vi "editDialog.vi"(0 "reference":refnum<class "ClassNode.lvclass">, 1 "insidePackageNode":bool, 5 "error in (no error)":errorcluster) -> (14 "reference out":refnum<class "ClassNode.lvclass">, 15 "changeConnection":T2, 16 "cancel":bool, 19 "error out":errorcluster)   [LabVIEW 2020, in "ClassNode.lvclass"]
doc: "Edit Dialog"
uses:
  <resource>/Framework/Providers/Open_GDS/UML/ClassNode_class/ClassNode.lvclass
  C:/Program Files (x86)/National Instruments/LabVIEW 2020/resource/Framework/Providers/Open_GDS/UML/AbstractNode_class/AbstractNode.lvclass
  <resource>/Framework/Providers/Open_GDS/UML/AbstractNode_class/private/NodeConnectionStatsType.ctl
  <resource>/Framework/Providers/Open_GDS/UML/UMLEditor/UMLEditor_StoredPathes.ctl
  <resource>/Framework/Providers/Open_GDS/ClassProviders/Common/CommonVIs/CommonVIs_StereoType.ctl
  <resource>/Framework/Providers/Open_GDS/UML/ContextHelp/ContextHelp_HelpTexts.ctl
  <resource>/Framework/Providers/Open_GDS/UML/MultiLineString_class/MultiLineString.lvclass
  <resource>/Framework/Providers/Open_GDS/UML/AbstractNode_class/AbstractNode.lvclass
  <resource>/Framework/Providers/Open_GDS/UML/Graph_class/Graph.lvclass
panel:
  in  "Class owner":u16(ring) items=["<No owner>"]
  out "RelText":string="Relative path used"
  out "UserText":string="When creating an enum-type just state the different enumeration members in a list like this:\nE.g.\nElement 1\nElement 2\n\nE.g.\nVolt(V)\nCurrent(A)\nResistance(ohm)\n"
  in  "ShowAttrib":bool caption="Show Attributes"
  in  "ShowMethods":bool caption="Show Methods"
  in  "Help":bool
  in  "AddMethod":bool
  in  "AddAttribute":bool
  in  "Stereo Type":T1(ring)=enum."ENUM"
  in  "Class Name":string
  in  "ClassPath":path caption="LvClassPath(Optional)"
  in  "Attribute":string
  in  "Methods":string
  in  "connection":bool caption="Connect to Package"
  in  "Cancel Button":bool
  in  "OK Button":bool
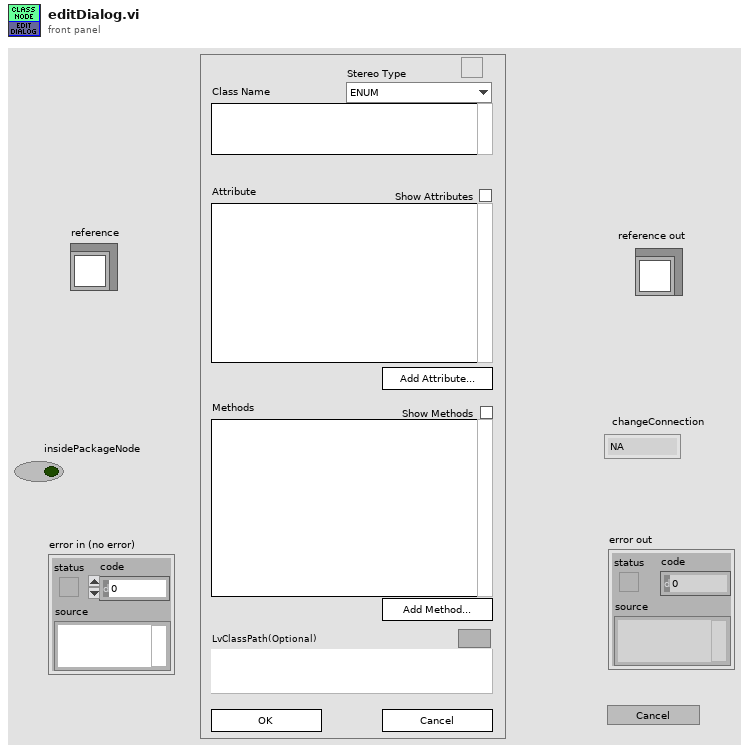
[diagram p1: front panel]
types:
  T1 = enum16{"None", "TYPE", "ENUM", "ABSTRACT", "ACTOR", "GUI", "SINGLETON", "SIGNAL", "BOUNDARY", "ENTITY", "CONTROL", "LEGACY", "APPLICATION", "VI", "LVLIB"}
  T2 = typedef "AbstractNode.lvclass/NodeConnectionStatsType.ctl" = enum16{"NA", "Connect", "DisConnect"}
  T3 = typedef "CommonVIs_StereoType.ctl" = enum16{"None", "TYPE", "ENUM", "ABSTRACT", "ACTOR", "GUI", "SINGLETON", "SIGNAL", "BOUNDARY", "ENTITY", "CONTROL", "LEGACY", "APPLICATION", "VI", "LVLIB", "INTERFACE"}
  T4 = typedef "UMLEditor_StoredPathes.ctl" = enum16{"LastSearchPath", "QueuedArrayStateVI", "ClassBasePath", "ViTemplatePath", "ApplicationTemplatePath", "IniFilePath", "WizDir", "RevPlugInPath"}
  T5 = enum32{"existing file", "new file", "new or existing file", "existing dir", "new dir", "new or existing dir", "existing file (use LLBs)", "new file (use LLBs)", "new or existing file (use LLBs)", "new or existing file or directory (use LLBs)"}
  T6 = enum16{"None", "TYPE", "ENUM", "GUI", "SINGLETON", "SIGNAL", "BOUNDARY", "ENTITY", "CONTROL", "LEGACY", "APPLICATION", "VI", "LVLIB"}
  T7 = typedef "ContextHelp_HelpTexts.ctl" = enum16{"None(Hide)", "Default", "Help", "Welcome", "GettingStarted", "ClassDiagram_Help", "SequenceDiagram_Help", "UseCaseDiagram_Help", "BSelect", "BClass", "BInterface", "BPackage", "BNote", "BDependency", "BInheritance", "BInterfaceImplementation", "BAssociation", "BAggregation", "BCompAggregation", "BNoteConnector", "BObject", "BActionBar", "BCall", "BSystem", "BActor", "BUseCase", "BGeneralization", "BIncludes", "BExtends", "BUseCaseDiagramAssociation", "ClassRelationshipEdge editDialog_Bent Style", "ClassRelationshipEdge editDialog_RelationType", "ClassRelationshipEdge editDialog_Reverse association", "ClassRelationshipEdge editDialog_Start label", "ClassRelationshipEdge editDialog_Middle label", "ClassRelationshipEdge editDialog_End label", "UMLEditor reversedEngineering_Pathes", "ReversedEngineering StateReverseDialog_Help", "ReversedEngineering StateQueuedSettings_Help", "UMLEditor reversedEngineering_AddTopVIs", "UMLEditor reversedEngineering_AddClasses", "UMLEditor reversedEngineering_AddDirs", "UMLEditor reversedEngineering_Recursively", "UMLEditor reversedEngineering_Remove", "UMLEditor reversedEngineering_ClearList", "UMLEditor reversedEngineering_HideSubAss", "UMLEditor reversedEngineering_CreateTypes", "UMLEditor reversedEngineering_OnlyInheritance", "UMLEditor reversedEngineering_CreateApplication", "UMLEditor reversedEngineering_OK", "UMLEditor reversedEngineering_Cancel", "UMLEditor reversedEngineering_Help", "UMLEditor createWizardScriptFile_ScriptfilePath", "UMLEditor createWizardScriptFile_ClassPath", "UMLEditor createWizardScriptFile_Use", "UMLEditor createWizardScriptFile_PrivateDirName", "UMLEditor createWizardScriptFile_DirAppend", "UMLEditor createWizardScriptFile_Separator Character", "UMLEditor createWizardScriptFile_OK", "UMLEditor createWizardScriptFile_Cancel", "UMLEditor createWizardScriptFile_Help", "ClassNode editDialog_Class Name", "InterfaceNode editDialog_Class Name", "ClassNode editDialog_Attribute", "ClassNode editDialog_Methods", "InterfaceNode editDialog_Methods", "ClassNode editDialog_connection", "InterfaceNode editDialog_connection", "ClassNode editDialog_StereoType", "ClassNode editDialog_ShowAttrib", "ClassNode editDialog_ShowMethods", "ClassNode editDialog_ClassPath", "ClassNode editDialog_AddAttribute", "ClassNode editDialog_AddMethod", "InterfaceNode editDialog_AddMethod", "ClassNode AttributeGuide_AttributeName", "ClassNode AttributeGuide_Array?", "ClassNode AttributeGuide_Data Type", "ClassNode AttributeGuide_RefName", "ClassNode AttributeGuide_Preview", "ClassNode AttributeGuide_OK", "ClassNode AttributeGuide_Cancel", "ClassNode MethodGuide_Visibility", "ClassNode MethodGuide_Method Name", "ClassNode MethodGuide_Preview", "ClassNode MethodGuide_OK", "ClassNode MethodGuide_Cancel", "CallNode EditCallProperties_AllButtons", "ObjectNode EditObjectlProperties_AllButtons", "ActorNode EditActorProperties_AllButtons", "UseCaseRelationshipNode EditUseCaselProperties_AllButtons", "UseCaseNode EditUseCaselProperties_AllButtons", "SystemNode EditSystemProperties_AllButtons", "ReversedEngineering UpdateAttributes_AllButtons", "StateNode editDialog_AllButtons", "StateTransition editDialog_AllButtons", "ArrangeNodes Main_Picture", "ArrangeNodes Main_Zoom", "ArrangeNodes Main_Auto Zoom", "ArrangeNodes Main_shorten", "ArrangeNodes Main_Min Length", "ArrangeNodes Main_Max Length", "ArrangeNodes Main_increase", "ArrangeNodes Main_decrease", "ArrangeNodes Main_Shake", "ArrangeNodes Main", "BState", "BInitialState", "BFinalState", "BStateTransition", "StateDiagram_Help", "StateDiagram_PropertiesAllButtons", "ReversedEngineering StateReverseDialog_ClearStates", "ReversedEngineering StateReverseDialog_UseQueuedStateMachines", "ReversedEngineering StateReverseDialog_QueuedSettings", "ReversedEngineering StateReverseDialog_SearchForVIs", "ReversedEngineering StateReverseDialog_SearchCriteria", "OptionsDialog_ClassBasePath", "OptionsDialog_VIPath", "OptionsDialog_ApplicationPath", "OptionsDialog_WizDir", "OptionsDialog_IniFilePath", "OptionsDialog_DefineColors", "OptionsDialog_Help", "OptionsDialog_CreateTypes", "ClassRelationshipEdge editDialog_SplitWire"}
  T8 = cluster{"Selection Start":u32, "Selection End":u32}
  T9 = typedef "ClassNode.lvclass/ObjectAttributes.ctl" = cluster{"midHeight":dbl, "botHeight":dbl, "name":refnum<class "MultiLineString.lvclass">, "attributes":refnum<class "MultiLineString.lvclass">, "methods":refnum<class "MultiLineString.lvclass">, "DEFAULT_COMPARTMENT_HEIGHT":i32, "DEFAULT_WIDTH":i32, "DEFAULT_HEIGHT":i32, "showMethods":bool, "showAttributes":bool, "ClassPath":path}
  T10 = typedef "AbstractNode.lvclass/ObjectAttributes.ctl" = cluster{"parent":refnum<class "AbstractNode.lvclass">, "children":refnum<class "AbstractNode.lvclass">[], "Hidden":bool}
  T11 = typedef "ContextHelp_ShowType.ctl" = cluster{"Header":string, "Picture":picture, "Text":string}
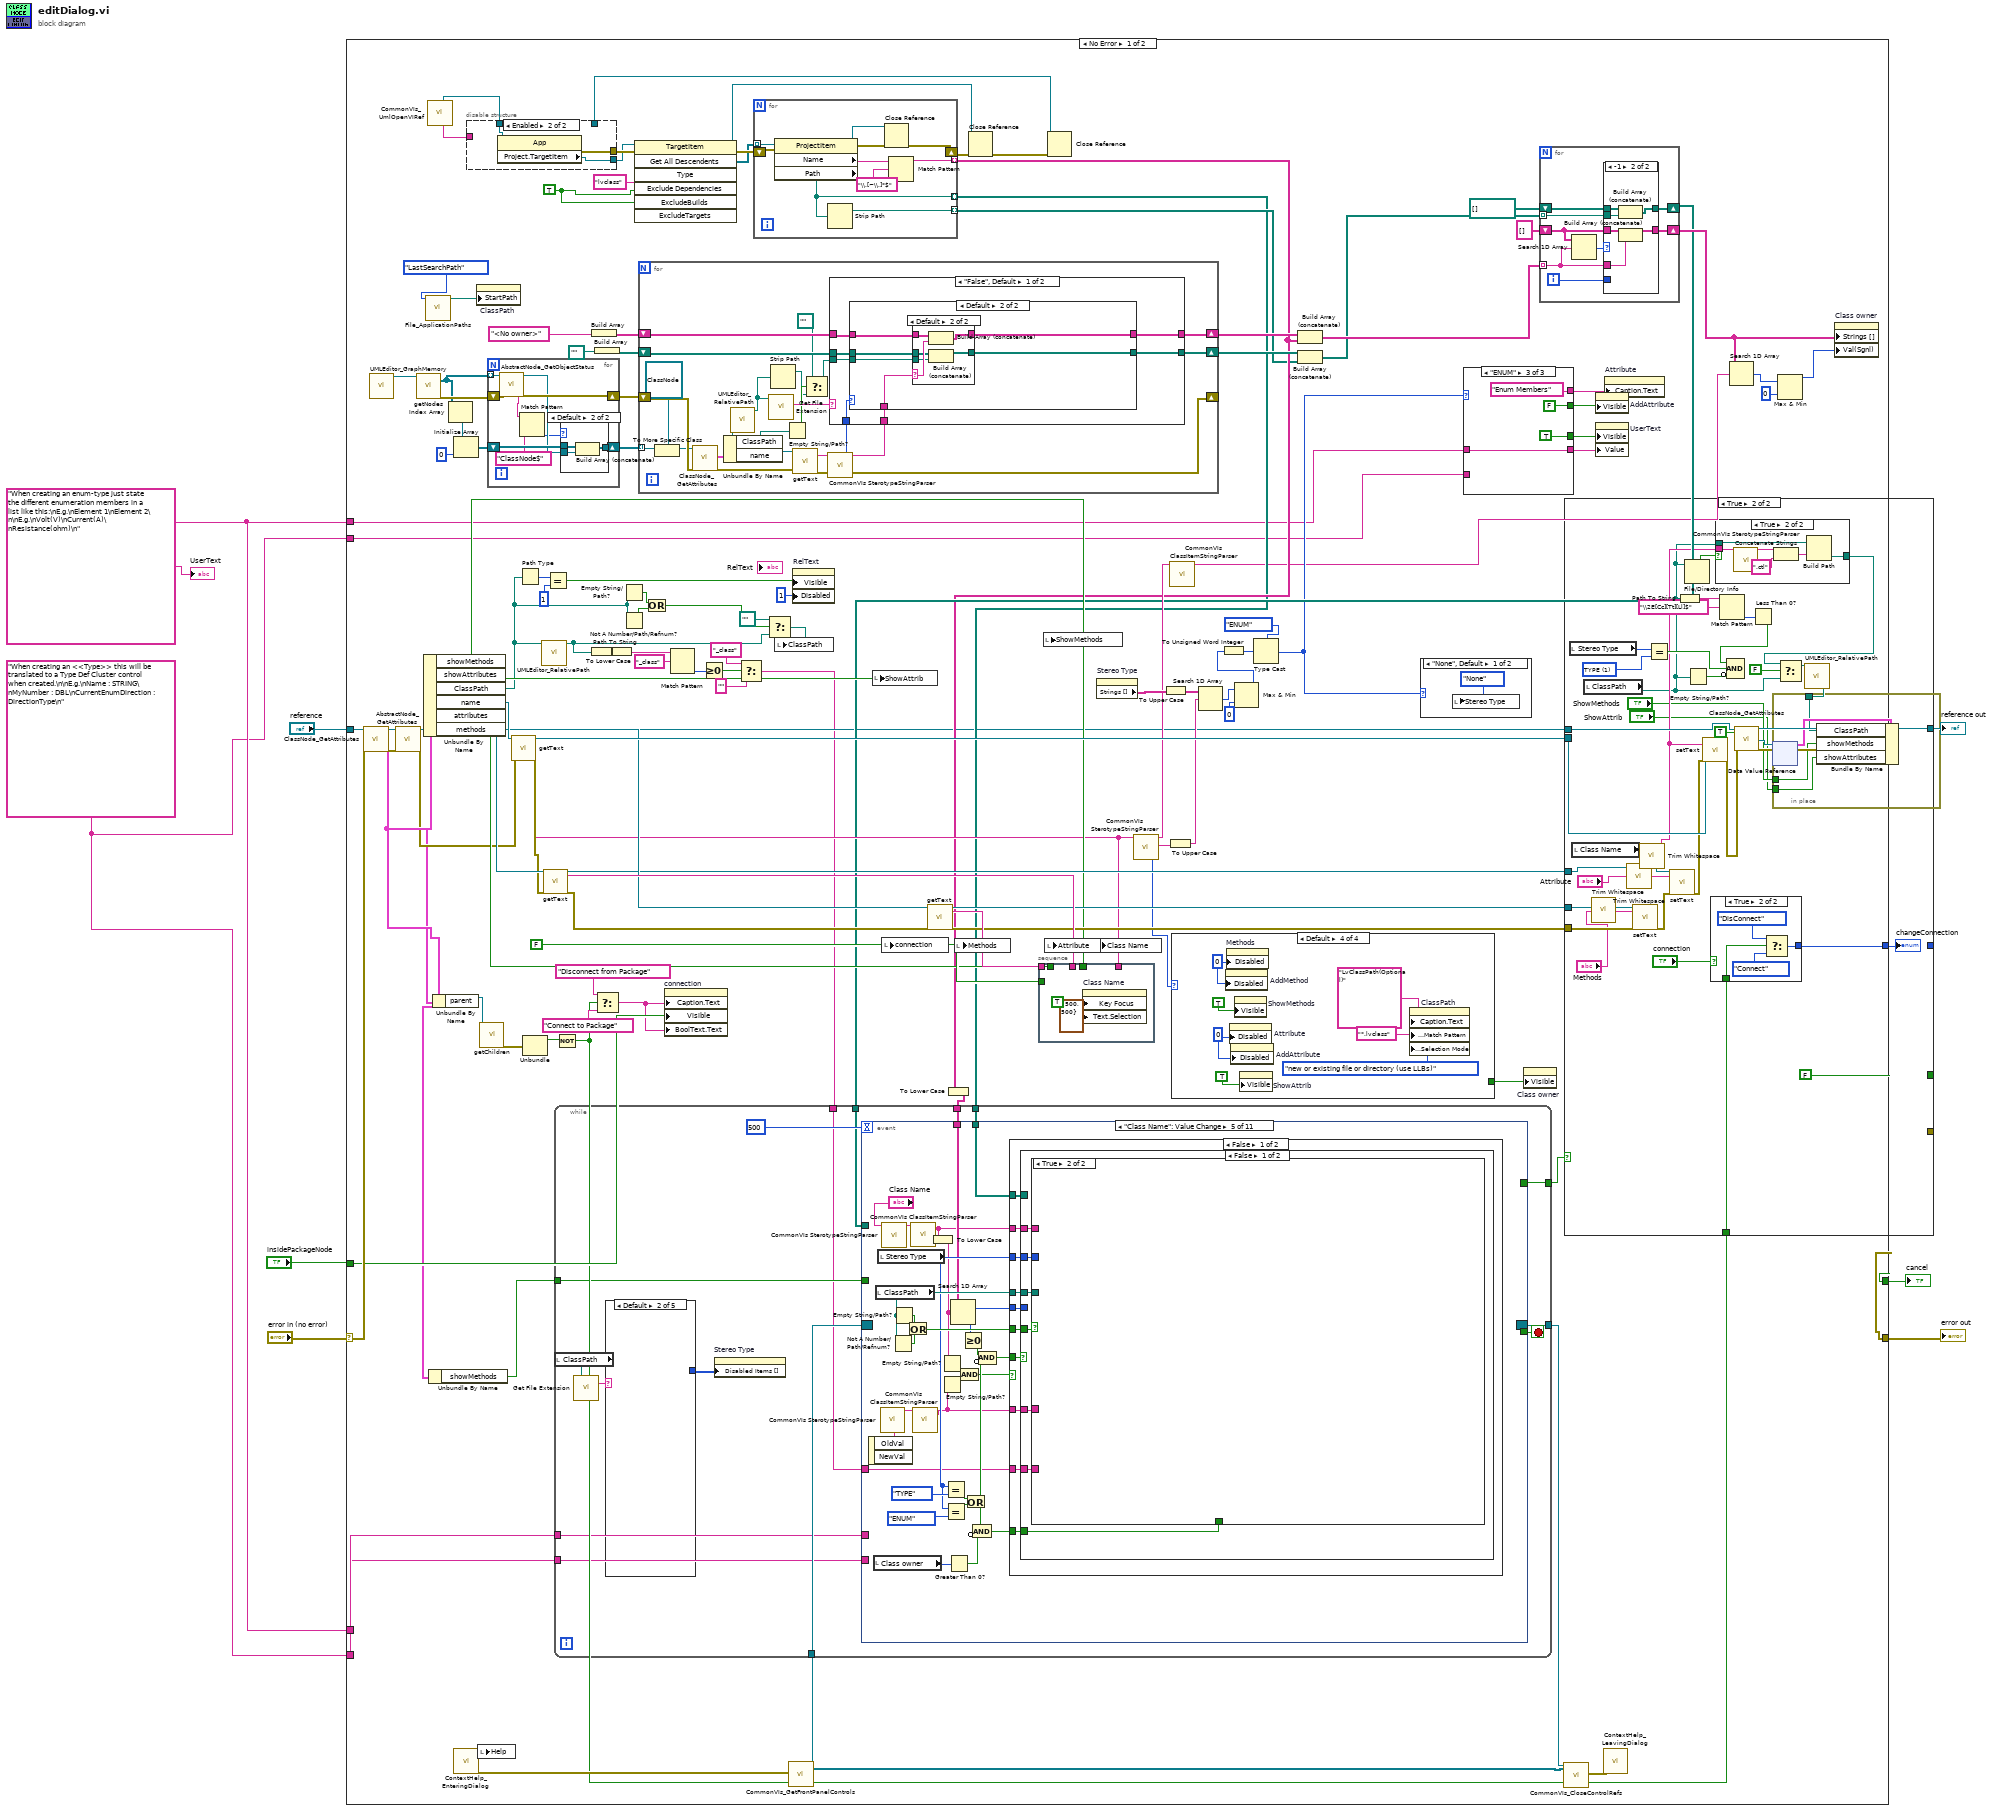
[diagram p0: block diagram]
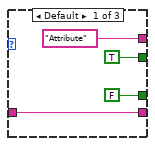
[diagram p2: hidden frame]
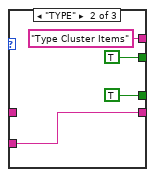
[diagram p3: hidden frame]
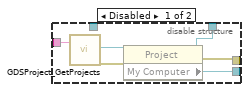
[diagram p4: hidden frame]
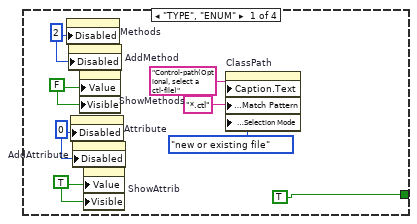
[diagram p10: hidden frame]
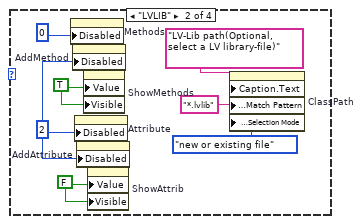
[diagram p11: hidden frame]
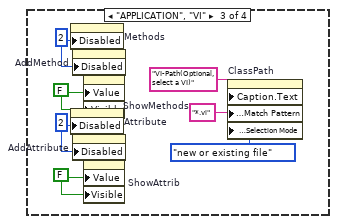
[diagram p12: hidden frame]
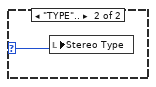
[diagram p13: hidden frame]
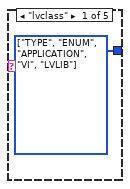
[diagram p14: hidden frame]
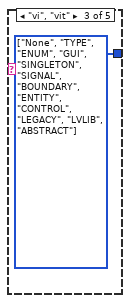
[diagram p15: hidden frame]
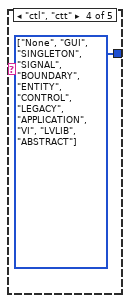
[diagram p16: hidden frame]
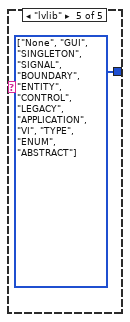
[diagram p17: hidden frame]
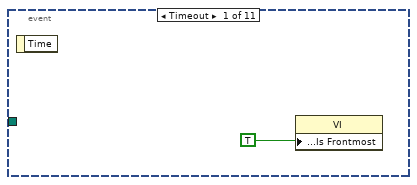
[diagram p18: hidden frame]
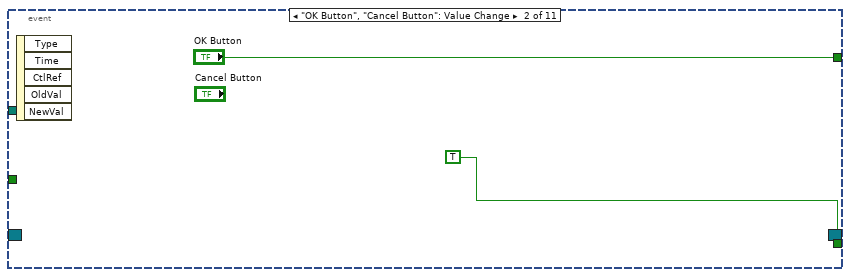
[diagram p19: hidden frame]
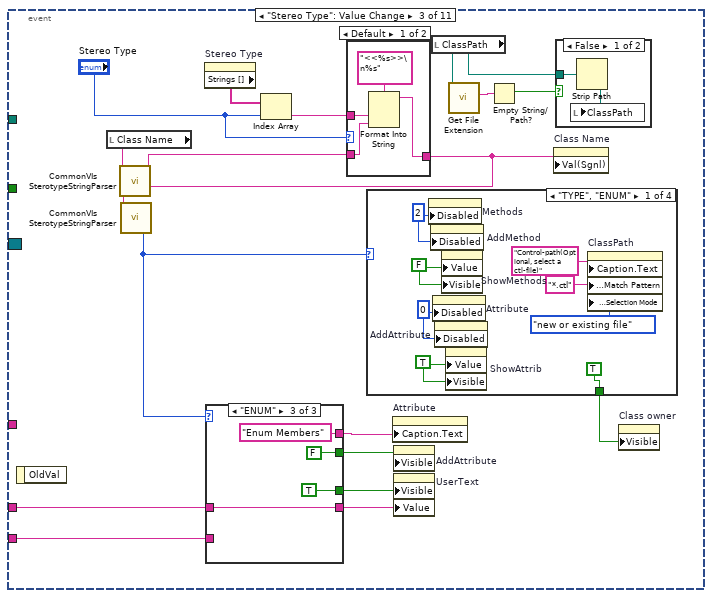
[diagram p20: hidden frame]
diagram:
  w1 = "When creating an <<Type>> this will be translated to a Type Def Cluster control when created.\n\nE.g.\nName : STRING\nMyNumber : DBL\nCurrentEnumDirection : DirectionType\n" ("UserText")
  w2 = "When creating an enum-type just state the different enumeration members in a list like this:\nE.g.\nElement 1\nElement 2\n\nE.g.\nVolt(V)\nCurrent(A)\nResistance(ohm)\n" ("UserText")
  n1 = case shown="No Error" "error in (no error)" {
    selector: "error in (no error)" -> [w131 w581]
    tunnel: "reference" -> [w132 w582]
    tunnel: [w134 w581] -> w7
    tunnel: [w133 w582] -> w6
    tunnel: "insidePackageNode" -> [w116 _]
    tunnel: [w114 _] -> w4
    tunnel: [w113 TRUE ("Key Focus")] -> w3
    tunnel: w2 -> [w22 _]
    tunnel: w1 -> [w21 _]
    tunnel: w2 -> [w29 _]
    tunnel: w1 -> [w28 _]
    frame No Error {
      w54 = TRUE ("ExcludeDependencies")
      w115 = FALSE ("connection")
      n2 = call <resource>:"ClassNode_GetAttributes.vi"("reference in"=w132, "error in (no error)"=w131) -> ("reference out"=w18:refnum<class "ClassNode.lvclass">, "Data"=w19:T9, "error out"=w17:errorcluster)  [unwired: 1 in, 14 out]
      n3 = call <resource>:"UMLEditor_GraphMemory.vi"() -> ("GraphOut"=w80:refnum<class "Graph.lvclass">)  [unwired: 2 in, 17 out]
      n4 = call <resource>:"AbstractNode_GetAttributes.vi"("reference in"=w18, "error in (no error)"=w17) -> ("reference out"=w15:refnum<class "ClassNode.lvclass">, "Data"=w14:T10, "error out"=w16:errorcluster)  [unwired: 14 in, 1 out]
      n5 = call-dynamic "getNodes.vi"("reference"=w80) -> ("nodes"=w79:refnum<class "AbstractNode.lvclass">[], "error out"=w84:errorcluster)  [unwired: 16 in, 1 out]
      n6 = Unbundle By Name(w19) -> ("showMethods"=w111:bool, "showAttributes"=w112:bool, "ClassPath"=w51:path, "name"=w128:refnum<class "MultiLineString.lvclass">, "attributes"=w127:refnum<class "MultiLineString.lvclass">, "methods"=w124:refnum<class "MultiLineString.lvclass">)
      n7 = call <resource>:"File_ApplicationPaths.vi"("PathName"=UMLEditor_StoredPathes."LastSearchPath" ("UMLPathes")) -> ("Path Out"=w91:path)  [unwired: 3 in, 15 out]
      n8 = call <resource>:"CommonVIs_UmlOpenVIRef.vi"() -> ("ProjectNameOut"=w74:string, "AppRefOut"=w35:refnum<vi>)  [unwired: 4 in, 6 out]
      n9 = Unbundle By Name(w19) -> ("showMethods"=w105:bool)
      n10 = Unbundle By Name(w14) -> ("parent"=w38:refnum<class "AbstractNode.lvclass">)
      n11 = Index Array(array=w79) -> (element=w83:refnum<class "AbstractNode.lvclass">)  [unwired: 1 in]
      n12 = Initialize Array(w83, 0 ("dimension size")) -> (w81:refnum<class "AbstractNode.lvclass">[])
      n13 = call <resource>:"ContextHelp_EnteringDialog.vi"() -> ("HelpStatus"=w104:bool, "error out"=w101:errorcluster)  [unwired: 3 in, 15 out]
      n14 = disable-structure shown="Enabled" {
        disable-tunnel: w74 -> [w150 _]
        disable-tunnel: [w149 w153] -> w72
        disable-tunnel: [w148 w154] -> w71
        disable-tunnel: [w147 _] -> w64
        disable-tunnel: w35 -> [_ w155]
        frame Disabled {
          n15 = call <resource>:"GDSProject_GetProjects.vi"("GetProjectRefByName"=w150) -> ("Project Refnum"=w152:refnum<vi>, "error out"=w151:errorcluster)  [unwired: 2 in, 15 out]
          n16 = property class="Project"(reference=w152, error in=w151) -> (reference out=w147:refnum<vi>, error out=w149:errorcluster, "My Computer"=w148:refnum<vi>)
        }
        frame Enabled {
          n17 = property class="App"(reference=w155) -> (error out=w153:errorcluster, "Project.TargetItem"=w154:refnum<vi>)  [unwired: 1 in, 1 out]
        }
      }
      n18 = property on="ClassPath" class="Path"("StartPath"=w91) -> ()  [unwired: 2 in, 2 out]
      n19 = local write "Help"(w104) -> ()
      n20 = call-dynamic "getChildren.vi"("reference"=w38) -> ("error out"=w40:errorcluster)  [unwired: 15 in, 3 out]
      n21 = for {
        shift-right: [w235] -> w77
        shift-left: w84 -> [w237]
        tunnel: w79 -> [w236] mode=indexing
        shift-right: [w232] -> w78
        shift-left: w81 -> [w234]
        n22 = call <resource>:"AbstractNode_GetObjectStatus.vi"("reference in"=w236, "error in (no error)"=w237) -> ("Class name"=w229:string, "reference out"=w233:refnum<class "AbstractNode.lvclass">, "error out"=w235:errorcluster)  [unwired: 15 out]
        n23 = Match Pattern(string=w229, regular expression="ClassNode$") -> (offset past match=w230:i32)  [unwired: 4 out]
        n24 = case shown="Default" w230 {
          tunnel: w234 -> [w238 w241]
          tunnel: w233 -> [_ w240]
          tunnel: [w238 w239] -> w232
          frame -1 {
          }
          frame Default {
            n25 = Build Array (concatenate)(w241, w240) -> (w239:refnum<class "AbstractNode.lvclass">[])
          }
        }
      }
      n26 = call-dynamic "getText.vi"("reference"=w128, "error in (no error)"=w16) -> ("reference out"=w130:refnum<class "MultiLineString.lvclass">, "text"=w110:string, "error out"=w123:errorcluster)  [unwired: 15 in]
      n27 = Path Type(1:w51) -> (0:w96:i16)
      n28 = Unbundle(w40) -> ("status"=w39:bool)  [unwired: 2 out]
      n29 = call <resource>:"UMLEditor_RelativePath.vi"("Path In"=w51) -> ("ConvertToAbsolutePath(If possible)"=w34:path)  [unwired: 1 in, 17 out]
      n30 = call-dynamic "getText.vi"("reference"=w127, "error in (no error)"=w123) -> ("reference out"=w121:refnum<class "MultiLineString.lvclass">, "text"=w126:string, "error out"=w122:errorcluster)  [unwired: 15 in]
      n31 = Equal?(x=w96, y=i16 1) -> (x = y?=w94:bool)
      n32 = Not(x=w39) -> (.not. x?=w37:bool)
      n33 = Path To String(path=w34) -> (string=w33:string)
      n34 = Build Array("<No owner>") -> (w75:string[])
      n35 = Build Array(path "" ("ClassPath")) -> (w63:path[])
      n36 = Select(t="Disconnect from Package", s=w37, f="Connect to Package") -> (s? t:f=w36:string)
      n37 = To Lower Case(string=w33) -> (all lower case string=w31:string)
      n38 = Not A Number/Path/Refnum?(number/path/refnum=w51) -> (NaN/Path/Refnum?=w53:bool)
      n39 = Empty String/Path?(string/path=w51) -> (empty?=w52:bool)
      n40 = invoke class="TargetItem" method="Get All Descendents"(reference=w71, error in=w72, "Type"="lvclass", "Exclude Dependencies"=w54, "ExcludeBuilds"=w54) -> (reference out=w67:refnum<vi>, error out=w69:errorcluster, "All Descendents"=w66:refnum<vi>[])  [unwired: 2 in, 4 out]
      n41 = for {
        tunnel: w78 -> [w185] mode=indexing
        shift-right: [w192] -> _
        shift-left: w77 -> [w203]
        shift-right: [w197] -> w70
        shift-left: w75 -> [w198]
        shift-right: [w193] -> w62
        shift-left: w63 -> [w194]
        n42 = To More Specific Class(target class=refnum<class "ClassNode.lvclass"> refnum ("reference in"), reference=w185) -> (specific class reference=w183:refnum<class "ClassNode.lvclass">)  [unwired: 1 in, 1 out]
        n43 = call <resource>:"ClassNode_GetAttributes.vi"("reference in"=w183, "error in (no error)"=w203) -> ("Data"=w182:T9, "error out"=w201:errorcluster)  [unwired: 1 in, 15 out]
        n44 = Unbundle By Name(w182) -> ("ClassPath"=w190:path, "name"=w202:refnum<class "MultiLineString.lvclass">)
        n45 = call <resource>:"UMLEditor_RelativePath.vi"("Path In"=w190) -> ("ConvertToAbsolutePath(If possible)"=w191:path)  [unwired: 1 in, 17 out]
        n46 = call <vilib>:"Get File Extension.vi"("file"=w191) -> ("lowercase file extension"=w199:string)  [unwired: 1 in, 9 out]
        n47 = Strip Path(path=w191) -> (stripped path=w188:path)  [unwired: 1 out]
        n48 = Empty String/Path?(string/path=w190) -> (empty?=w189:bool)
        n49 = call-dynamic "getText.vi"("reference"=w202, "error in (no error)"=w201) -> ("text"=w200:string, "error out"=w192:errorcluster)  [unwired: 15 in, 1 out]
        n50 = Select(t=path "", s=w189, f=w188) -> (s? t:f=w187:path)
        n51 = call <resource>:"CommonVIs SterotypeStringParser.vi"("SterotypeStringIn"=w200) -> ("StereoType"=w196:T3, "Name"=w195:string)  [unwired: 17 out]
        n52 = case shown="\"False\", Default" w199 {
          tunnel: w198 -> [w209 w228]
          tunnel: [w210 w228] -> w197
          tunnel: w196 -> [w208 _]
          tunnel: w195 -> [w207 _]
          tunnel: w194 -> [w206 w227]
          tunnel: [w205 w227] -> w193
          tunnel: w187 -> [w204 _]
          frame "False", Default {
            n53 = case shown="Default" w208 {
              tunnel: [w212 w218] -> w210
              tunnel: w209 -> [w212 w217]
              tunnel: w207 -> [_ w216]
              tunnel: w206 -> [w211 w215]
              tunnel: [w211 w214] -> w205
              tunnel: w204 -> [_ w213]
              frame "TYPE", "ENUM", "APPLICATION".."LVLIB" {
              }
              frame Default {
                n54 = case shown="Default" w216 {
                  selector: w216 -> [_ w225]
                  tunnel: [w220 w224] -> w218
                  tunnel: w217 -> [w220 w226]
                  tunnel: w215 -> [w219 w223]
                  tunnel: [w219 w222] -> w214
                  tunnel: w213 -> [_ w221]
                  frame "" {
                  }
                  frame Default {
                    n55 = Build Array (concatenate)(w226, w225) -> (w224:string[])
                    n56 = Build Array (concatenate)(w223, w221) -> (w222:path[])
                  }
                }
              }
            }
          }
          frame "ctl", "ctt", "vi", "vit" {
          }
        }
      }
      n57 = Or(x=w52, y=w53) -> (x .or. y?=w50:bool)
      n58 = property on="connection" class="Bool (strict)"("Caption.Text"=w36, "Visible"=w116, "BoolText.Text"=w36) -> ()  [unwired: 2 in, 2 out]
      n59 = Match Pattern(string=w31, regular expression="_class") -> (offset past match=w30:i32)  [unwired: 1 in, 3 out]
      n60 = Greater Or Equal To 0?(x=w30) -> (x >= 0?=w13:bool)
      n61 = Select(t="_class" ("regular expression"), s=w13, f="") -> (s? t:f=w11:string)
      n62 = for {
        tunnel: w66 -> [w181] mode=indexing
        tunnel: [w178] -> w44 mode=indexing
        shift-right: [w174] -> w68
        shift-left: w69 -> [w175]
        tunnel: [w173] -> w42 mode=indexing
        tunnel: [w172] -> w41 mode=indexing
        n63 = property class="ProjectItem"(reference=w181, error in=w175) -> (reference out=w176:refnum<vi>, error out=w177:errorcluster, "Name"=w180:string, "Path"=w172:path)
        n64 = Strip Path(path=w172) -> (stripped path=w173:path)  [unwired: 1 out]
        n65 = Close Reference(reference=w176, error in (no error)=w177) -> (error out=w174:errorcluster)
        n66 = Match Pattern(string=w180, regular expression="\\.[~\\.]*$") -> (before substring=w178:string)  [unwired: 4 out]
      }
      n67 = Select(t=path "", s=w50, f=w34) -> (s? t:f=w93:path)
      n68 = local write "ClassPath"(w93) -> ()
      n69 = call <resource>:"CommonVIs_GetFrontPanelControls.vi"("error in (no error)"=w101) -> ("Event Registration Refnum"=w100:refnum<event-registration>, "ControlRefs"=w103:refnum<vi>[])  [unwired: 1 in, 16 out]
      n70 = property on="RelText" class="Str"("Visible"=w94, "Disabled"=u8 1) -> ()  [unwired: 2 in, 2 out]
      n71 = local write "ShowAttrib"(w112) -> ()
      n72 = local write "connection"(w115) -> ()
      n73 = call-dynamic "getText.vi"("reference"=w124, "error in (no error)"=w122) -> ("reference out"=w120:refnum<class "MultiLineString.lvclass">, "text"=w125:string, "error out"=w119:errorcluster)  [unwired: 15 in]
      n74 = To Lower Case(string=w44) -> (all lower case string=w47:string[])
      n75 = local write "Methods"(w125) -> ()
      n76 = Close Reference(reference=w67, error in (no error)=w68) -> (error out=w65:errorcluster)
      n77 = stacked-sequence {
        tunnel: w110 -> [_]
        tunnel: w125 -> [_]
        tunnel: w115 -> [_]
        tunnel: w126 -> [_]
        tunnel: w112 -> [_]
        tunnel: w111 -> [_]
        frame #0 {
          n78 = property on="Class Name" class="Str"("Key Focus"=TRUE, "Text.Selection"=T8 {"Selection Start"=500, "Selection End"=500}) -> ()  [unwired: 2 in, 2 out]
        }
      }
      n79 = local write "ShowMethods"(w111) -> ()
      n80 = local write "Attribute"(w126) -> ()
      n81 = Close Reference(reference=w64, error in (no error)=w65) -> ()  [unwired: 1 out]
      n82 = local write "Class Name"(w110) -> ()
      n83 = property on="Stereo Type" class="Enum (strict)"() -> ("Strings []"=w108:string[])  [unwired: 2 in, 2 out]
      n84 = call <resource>:"CommonVIs SterotypeStringParser.vi"("SterotypeStringIn"=w110) -> ("StereoType"=w98:T3, "Name"=w61:string, "Sterotype"=w109:string)  [unwired: 16 out]
      n85 = To Upper Case(1:w108) -> (0:w107:string[])
      n86 = To Upper Case(1:w109) -> (0:w106:string)
      n87 = call <resource>:"CommonVIs ClassItemStringParser.vi"("ClassItemNameIn"=w61) -> ("Class"=w20:string)  [unwired: 18 out]
      n88 = case shown="Default" w98 {
        tunnel: [TRUE ("ShowMethods") _ _ _] -> w85
        frame "TYPE", "ENUM" {
          w246 = TRUE ("ShowMethods")
          w247 = u8 0 ("Disabled")
          w248 = FALSE ("ShowMethods")
          w249 = u8 2 ("Disabled")
          n89 = property on="Methods" class="Str"("Disabled"=w249) -> ()  [unwired: 2 in, 2 out]
          n90 = property on="AddMethod" class="Bool"("Disabled"=w249) -> ()  [unwired: 2 in, 2 out]
          n91 = property on="Attribute" class="Str"("Disabled"=w247) -> ()  [unwired: 2 in, 2 out]
          n92 = property on="AddAttribute" class="Bool"("Disabled"=w247) -> ()  [unwired: 2 in, 2 out]
          n93 = property on="ShowMethods" class="Bool (strict)"("Value"=w248, "Visible"=w248) -> ()  [unwired: 2 in, 2 out]
          n94 = property on="ShowAttrib" class="Bool (strict)"("Value"=w246, "Visible"=w246) -> ()  [unwired: 2 in, 2 out]
          n95 = property on="ClassPath" class="Path"("Caption.Text"="Control-path(Optional, select a ctl-file)", "Browse Options:Match Pattern"="*.ctl" ("Browse Dialog Options:Pattern Label"), "Browse Options:Selection Mode"=T5."new or existing file" ("Browse Dialog Options:Selection Mode")) -> ()  [unwired: 2 in, 2 out]
        }
        frame "LVLIB" {
          w254 = FALSE ("ShowMethods")
          w251 = u8 2 ("Disabled")
          w255 = TRUE ("ShowMethods")
          n96 = property on="Methods" class="Str"("Disabled"=u8 0) -> ()  [unwired: 2 in, 2 out]
          n97 = property on="AddMethod" class="Bool"("Disabled"=w251) -> ()  [unwired: 2 in, 2 out]
          n98 = property on="Attribute" class="Str"("Disabled"=w251) -> ()  [unwired: 2 in, 2 out]
          n99 = property on="AddAttribute" class="Bool"("Disabled"=w251) -> ()  [unwired: 2 in, 2 out]
          n100 = property on="ShowMethods" class="Bool (strict)"("Value"=w255, "Visible"=w255) -> ()  [unwired: 2 in, 2 out]
          n101 = property on="ShowAttrib" class="Bool (strict)"("Value"=w254, "Visible"=w254) -> ()  [unwired: 2 in, 2 out]
          n102 = property on="ClassPath" class="Path"("Caption.Text"="LV-Lib path(Optional, select a LV library-file)", "Browse Options:Match Pattern"="*.lvlib" ("Browse Dialog Options:Pattern Label"), "Browse Options:Selection Mode"=T5."new or existing file" ("Browse Dialog Options:Selection Mode")) -> ()  [unwired: 2 in, 2 out]
        }
        frame "APPLICATION", "VI" {
          w260 = FALSE ("ShowMethods")
          w262 = u8 2 ("Disabled")
          w261 = FALSE ("ShowMethods")
          w263 = u8 2 ("Disabled")
          n103 = property on="Methods" class="Str"("Disabled"=w263) -> ()  [unwired: 2 in, 2 out]
          n104 = property on="Attribute" class="Str"("Disabled"=w262) -> ()  [unwired: 2 in, 2 out]
          n105 = property on="AddMethod" class="Bool"("Disabled"=w263) -> ()  [unwired: 2 in, 2 out]
          n106 = property on="AddAttribute" class="Bool"("Disabled"=w262) -> ()  [unwired: 2 in, 2 out]
          n107 = property on="ShowMethods" class="Bool (strict)"("Value"=w261, "Visible"=w261) -> ()  [unwired: 2 in, 2 out]
          n108 = property on="ShowAttrib" class="Bool (strict)"("Value"=w260, "Visible"=w260) -> ()  [unwired: 2 in, 2 out]
          n109 = property on="ClassPath" class="Path"("Caption.Text"="VI-Path(Optional, select a VI)", "Browse Options:Match Pattern"="*.vi" ("Browse Dialog Options:Pattern Label"), "Browse Options:Selection Mode"=T5."new or existing file" ("Browse Dialog Options:Selection Mode")) -> ()  [unwired: 2 in, 2 out]
        }
        frame Default {
          w269 = u8 0 ("Disabled")
          w270 = u8 0 ("Disabled")
          n110 = property on="AddMethod" class="Bool"("Disabled"=w270) -> ()  [unwired: 2 in, 2 out]
          n111 = property on="Methods" class="Str"("Disabled"=w270) -> ()  [unwired: 2 in, 2 out]
          n112 = property on="Attribute" class="Str"("Disabled"=w269) -> ()  [unwired: 2 in, 2 out]
          n113 = property on="AddAttribute" class="Bool"("Disabled"=w269) -> ()  [unwired: 2 in, 2 out]
          n114 = property on="ShowMethods" class="Bool (strict)"("Visible"=TRUE ("ShowMethods")) -> ()  [unwired: 2 in, 2 out]
          n115 = property on="ShowAttrib" class="Bool (strict)"("Visible"=TRUE ("ShowMethods")) -> ()  [unwired: 2 in, 2 out]
          n116 = property on="ClassPath" class="Path"("Caption.Text"="LvClassPath(Optional)", "Browse Options:Match Pattern"="*.lvclass" ("Browse Dialog Options:Pattern Label"), "Browse Options:Selection Mode"=T5."new or existing file or directory (use LLBs)" ("Browse Dialog Options:Selection Mode")) -> ()  [unwired: 2 in, 2 out]
        }
      }
      n117 = Search 1D Array(1D array=w107, element=w106) -> (index of element=w87:i32)  [unwired: 1 out]
      n118 = Max & Min(x=w87, y=0) -> (max(x,y)=w86:i32)  [unwired: 1 out]
      n119 = To Unsigned Word Integer(number=w86) -> (unsigned 16bit integer=w90:u16)
      n120 = Type Cast(type=CommonVIs_StereoType."ENUM" ("StereoType"), x=w90) -> (*(type *) &x=w23:T3)
      n121 = Build Array (concatenate)(w70, w44) -> (w45:string[])
      n122 = Build Array (concatenate)(w62, w42) -> (w43:path[])
      n123 = case shown="\"None\", Default" w23 {
        selector: w23 -> [_ w272]
        frame "None", Default {
          n124 = local write "Stereo Type"(CommonVIs_StereoType."None" ("StereoType")) -> ()
        }
        frame "TYPE".. {
          n125 = local write "Stereo Type"(w272) -> ()
        }
      }
      n126 = case shown="\"ENUM\"" w23 {
        tunnel: ["Attribute" ("Caption.Text") "Type Cluster Items" ("Caption.Text") "Enum Members" ("Caption.Text")] -> w24
        tunnel: [TRUE ("Key Focus") TRUE ("Key Focus") FALSE ("Key Focus")] -> w27
        tunnel: [FALSE ("Key Focus") TRUE ("Key Focus") TRUE ("Key Focus")] -> w25
        tunnel: [w135 w139 w143] -> w26
        tunnel: w22 -> [w135 _ w143]
        tunnel: w21 -> [_ w139 _]
        frame Default {
        }
        frame "TYPE" {
        }
        frame "ENUM" {
        }
      }
      n127 = property on="Class owner" class="Ring (strict)"("Visible"=w85) -> ()  [unwired: 2 in, 2 out]
      n128 = for {
        tunnel: w45 -> [w162] mode=indexing
        shift-right: [w161] -> w57
        shift-left: string[] [] -> [w160]
        shift-right: [w158] -> w46
        shift-left: path[] [] -> [w157]
        tunnel: w43 -> [w156] mode=indexing
        i -> [w159]
        n129 = Search 1D Array(1D array=w160, element=w162) -> (index of element=w163:i32)  [unwired: 1 out]
        n130 = case shown="-1" w163 {
          tunnel: w162 -> [_ w171]
          tunnel: [w165 w169] -> w161
          tunnel: w160 -> [w165 w170]
          tunnel: w159 -> [_ _]
          tunnel: [w164 w167] -> w158
          tunnel: w157 -> [w164 w168]
          tunnel: w156 -> [_ w166]
          frame Default {
          }
          frame -1 {
            n131 = Build Array (concatenate)(w168, w166) -> (w167:path[])
            n132 = Build Array (concatenate)(w170, w171) -> (w169:string[])
          }
        }
      }
      n133 = while {
        tunnel: [w287] -> w129
        tunnel: w105 -> [w285]
        tunnel: w100 -> [w283]
        tunnel: [w282] -> w99
        tunnel: w46 -> [w278]
        tunnel: w47 -> [w277]
        tunnel: w41 -> [w276]
        tunnel: w11 -> [w275]
        tunnel: w29 -> [w274]
        tunnel: w28 -> [w273]
        stop <- w286 stop-if-true
        n134 = local read "ClassPath"() -> (w281:path)
        n135 = call <vilib>:"Get File Extension.vi"("file"=w281) -> ("lowercase file extension"=w280:string)  [unwired: 1 in, 9 out]
        n136 = case shown="Default" w280 {
          tunnel: [w288 _ w289 w290 w291] -> w279
          frame "lvclass" {
            w288 = T3[] [enum."TYPE", enum."ENUM", enum."APPLICATION", enum."VI", enum."LVLIB"] items=["None", "TYPE", "ENUM", "ABSTRACT", "ACTOR", "GUI", "SINGLETON", "SIGNAL", "BOUNDARY", "ENTITY", "CONTROL", "LEGACY", "APPLICATION", "VI", "LVLIB", "INTERFACE"] ("Disabled Items []")
          }
          frame Default {
          }
          frame "vi", "vit" {
            w289 = T3[] [enum."None", enum."TYPE", enum."ENUM", enum."GUI", enum."SINGLETON", enum."SIGNAL", enum."BOUNDARY", enum."ENTITY", enum."CONTROL", enum."LEGACY", enum."LVLIB", enum."ABSTRACT"] items=["None", "TYPE", "ENUM", "ABSTRACT", "ACTOR", "GUI", "SINGLETON", "SIGNAL", "BOUNDARY", "ENTITY", "CONTROL", "LEGACY", "APPLICATION", "VI", "LVLIB", "INTERFACE"] ("Disabled Items []")
          }
          frame "ctl", "ctt" {
            w290 = T3[] [enum."None", enum."GUI", enum."SINGLETON", enum."SIGNAL", enum."BOUNDARY", enum."ENTITY", enum."CONTROL", enum."LEGACY", enum."APPLICATION", enum."VI", enum."LVLIB", enum."ABSTRACT"] items=["None", "TYPE", "ENUM", "ABSTRACT", "ACTOR", "GUI", "SINGLETON", "SIGNAL", "BOUNDARY", "ENTITY", "CONTROL", "LEGACY", "APPLICATION", "VI", "LVLIB", "INTERFACE"] ("Disabled Items []")
          }
          frame "lvlib" {
            w291 = T3[] [enum."None", enum."GUI", enum."SINGLETON", enum."SIGNAL", enum."BOUNDARY", enum."ENTITY", enum."CONTROL", enum."LEGACY", enum."APPLICATION", enum."VI", enum."TYPE", enum."ENUM", enum."ABSTRACT"] items=["None", "TYPE", "ENUM", "ABSTRACT", "ACTOR", "GUI", "SINGLETON", "SIGNAL", "BOUNDARY", "ENTITY", "CONTROL", "LEGACY", "APPLICATION", "VI", "LVLIB", "INTERFACE"] ("Disabled Items []")
          }
        }
        n137 = property on="Stereo Type" class="Enum (strict)"("Disabled Items []"=w279) -> ()  [unwired: 2 in, 2 out]
        n138 = event shown="[4] \"Class Name\": Value Change" {
          selector: w283 -> [_ _ _ _ _ _ _ _ _ _ _]
          dyn-events: [_ _ _ _ _ _ _ _ _ _ _] -> w282
          timeout: 500 -> [_ _ _ _ _ _ _ _ _ _ _]
          tunnel: [_ "OK Button" _ FALSE ("OK Button") _ _ _ _ _ _ _] -> w287
          tunnel: [_ TRUE _ TRUE _ _ _ _ _ _ _] -> w286
          tunnel: w285 -> [_ _ _ _ _ _ _ _ _ _ _]
          tunnel: w278 -> [_ _ _ _ _ _ w442 _ _ _ _]
          tunnel: w277 -> [_ _ _ _ w375 _ _ _ _ _ _]
          tunnel: w276 -> [_ _ _ _ w370 _ _ _ _ _ _]
          tunnel: w275 -> [_ _ _ _ w369 _ _ _ _ _ _]
          tunnel: w274 -> [_ _ w296 _ _ _ _ _ _ _ _]
          tunnel: w273 -> [_ _ w295 _ _ _ _ _ _ _ _]
          event Timeout {
            n139 = event-data() -> ()  [unwired: 2 out]
            n140 = property class="VI"("Front Panel Window:Is Frontmost"=TRUE) -> ()  [unwired: 2 in, 2 out]
          }
          event "OK Button", "Cancel Button": Value Change {
            n141 = event-data() -> ()  [unwired: 6 out]
          }
          event "Stereo Type": Value Change {
            n142 = event-data() -> ()  [unwired: 2 out]
            n143 = local read "Class Name"() -> (w306:string)
            n144 = call <resource>:"CommonVIs SterotypeStringParser.vi"("SterotypeStringIn"=w306) -> ("Name"=w310:string)  [unwired: 18 out]
            n145 = property on="Stereo Type" class="Enum (strict)"() -> ("Strings []"=w311:string[])  [unwired: 2 in, 2 out]
            n146 = Index Array(array=w311, index="Stereo Type") -> (element=w305:string)
            n147 = case shown="Default" "Stereo Type" {
              tunnel: w305 -> [w357 _]
              tunnel: w310 -> [w356 w359]
              tunnel: [w355 w359] -> w303
              frame Default {
                n148 = Format Into String(format string="<<%s>>\n%s", w357, w356) -> (resulting string=w355:string)  [unwired: 2 in, 1 out]
              }
              frame "None" {
              }
            }
            n149 = call <resource>:"CommonVIs SterotypeStringParser.vi"("SterotypeStringIn"=w303) -> ("StereoType"=w299:T3)  [unwired: 18 out]
            n150 = case shown="\"ENUM\"" w299 {
              tunnel: ["Attribute" ("Caption.Text") "Type Cluster Items" ("Caption.Text") "Enum Members" ("Caption.Text")] -> w309
              tunnel: [TRUE ("Key Focus") TRUE ("Key Focus") FALSE ("Key Focus")] -> w308
              tunnel: [FALSE ("Key Focus") TRUE ("Key Focus") TRUE ("Key Focus")] -> w307
              tunnel: [w343 w347 w351] -> w297
              tunnel: w296 -> [w343 _ w351]
              tunnel: w295 -> [_ w347 _]
              frame Default {
              }
              frame "TYPE" {
              }
              frame "ENUM" {
              }
            }
            n151 = case shown="\"TYPE\", \"ENUM\"" w299 {
              tunnel: [TRUE ("ShowMethods") _ _ _] -> w298
              frame "TYPE", "ENUM" {
                w316 = TRUE ("ShowMethods")
                w317 = u8 0 ("Disabled")
                w318 = FALSE ("ShowMethods")
                w319 = u8 2 ("Disabled")
                n152 = property on="Methods" class="Str"("Disabled"=w319) -> ()  [unwired: 2 in, 2 out]
                n153 = property on="AddMethod" class="Bool"("Disabled"=w319) -> ()  [unwired: 2 in, 2 out]
                n154 = property on="Attribute" class="Str"("Disabled"=w317) -> ()  [unwired: 2 in, 2 out]
                n155 = property on="AddAttribute" class="Bool"("Disabled"=w317) -> ()  [unwired: 2 in, 2 out]
                n156 = property on="ShowMethods" class="Bool (strict)"("Value"=w318, "Visible"=w318) -> ()  [unwired: 2 in, 2 out]
                n157 = property on="ShowAttrib" class="Bool (strict)"("Value"=w316, "Visible"=w316) -> ()  [unwired: 2 in, 2 out]
                n158 = property on="ClassPath" class="Path"("Caption.Text"="Control-path(Optional, select a ctl-file)", "Browse Options:Match Pattern"="*.ctl" ("Browse Dialog Options:Pattern Label"), "Browse Options:Selection Mode"=T5."new or existing file" ("Browse Dialog Options:Selection Mode")) -> ()  [unwired: 2 in, 2 out]
              }
              frame "LVLIB" {
                w324 = FALSE ("ShowMethods")
                w321 = u8 2 ("Disabled")
                w325 = TRUE ("ShowMethods")
                n159 = property on="Methods" class="Str"("Disabled"=u8 0) -> ()  [unwired: 2 in, 2 out]
                n160 = property on="AddMethod" class="Bool"("Disabled"=w321) -> ()  [unwired: 2 in, 2 out]
                n161 = property on="Attribute" class="Str"("Disabled"=w321) -> ()  [unwired: 2 in, 2 out]
                n162 = property on="AddAttribute" class="Bool"("Disabled"=w321) -> ()  [unwired: 2 in, 2 out]
                n163 = property on="ShowMethods" class="Bool (strict)"("Value"=w325, "Visible"=w325) -> ()  [unwired: 2 in, 2 out]
                n164 = property on="ShowAttrib" class="Bool (strict)"("Value"=w324, "Visible"=w324) -> ()  [unwired: 2 in, 2 out]
                n165 = property on="ClassPath" class="Path"("Caption.Text"="LV-Lib path(Optional, select a LV library-file)", "Browse Options:Match Pattern"="*.lvlib" ("Browse Dialog Options:Pattern Label"), "Browse Options:Selection Mode"=T5."new or existing file" ("Browse Dialog Options:Selection Mode")) -> ()  [unwired: 2 in, 2 out]
              }
              frame "APPLICATION", "VI" {
                w330 = FALSE ("ShowMethods")
                w332 = u8 2 ("Disabled")
                w331 = FALSE ("ShowMethods")
                w333 = u8 2 ("Disabled")
                n166 = property on="Methods" class="Str"("Disabled"=w333) -> ()  [unwired: 2 in, 2 out]
                n167 = property on="Attribute" class="Str"("Disabled"=w332) -> ()  [unwired: 2 in, 2 out]
                n168 = property on="AddMethod" class="Bool"("Disabled"=w333) -> ()  [unwired: 2 in, 2 out]
                n169 = property on="AddAttribute" class="Bool"("Disabled"=w332) -> ()  [unwired: 2 in, 2 out]
                n170 = property on="ShowMethods" class="Bool (strict)"("Value"=w331, "Visible"=w331) -> ()  [unwired: 2 in, 2 out]
                n171 = property on="ShowAttrib" class="Bool (strict)"("Value"=w330, "Visible"=w330) -> ()  [unwired: 2 in, 2 out]
                n172 = property on="ClassPath" class="Path"("Caption.Text"="VI-Path(Optional, select a VI)", "Browse Options:Match Pattern"="*.vi" ("Browse Dialog Options:Pattern Label"), "Browse Options:Selection Mode"=T5."new or existing file" ("Browse Dialog Options:Selection Mode")) -> ()  [unwired: 2 in, 2 out]
              }
              frame Default {
                w337 = TRUE ("ShowMethods")
                w339 = u8 0 ("Disabled")
                w338 = TRUE ("ShowMethods")
                w340 = u8 0 ("Disabled")
                n173 = property on="AddMethod" class="Bool"("Disabled"=w340) -> ()  [unwired: 2 in, 2 out]
                n174 = property on="Methods" class="Str"("Disabled"=w340) -> ()  [unwired: 2 in, 2 out]
                n175 = property on="Attribute" class="Str"("Disabled"=w339) -> ()  [unwired: 2 in, 2 out]
                n176 = property on="AddAttribute" class="Bool"("Disabled"=w339) -> ()  [unwired: 2 in, 2 out]
                n177 = property on="ShowMethods" class="Bool (strict)"("Value"=w338, "Visible"=w338) -> ()  [unwired: 2 in, 2 out]
                n178 = property on="ShowAttrib" class="Bool (strict)"("Value"=w337, "Visible"=w337) -> ()  [unwired: 2 in, 2 out]
                n179 = property on="ClassPath" class="Path"("Caption.Text"="LvClassPath(Optional)", "Browse Options:Match Pattern"="*.lvclass" ("Browse Dialog Options:Pattern Label"), "Browse Options:Selection Mode"=T5."new or existing file or directory (use LLBs)" ("Browse Dialog Options:Selection Mode")) -> ()  [unwired: 2 in, 2 out]
              }
            }
            n180 = property on="Attribute" class="Str"("Caption.Text"=w309) -> ()  [unwired: 2 in, 2 out]
            n181 = property on="AddAttribute" class="Bool"("Visible"=w308) -> ()  [unwired: 2 in, 2 out]
            n182 = property on="UserText" class="Str"("Visible"=w307, "Value"=w297) -> ()  [unwired: 2 in, 2 out]
            n183 = local read "ClassPath"() -> (w300:path)
            n184 = call <vilib>:"Get File Extension.vi"("file"=w300) -> ("lowercase file extension"=w302:string)  [unwired: 1 in, 9 out]
            n185 = Empty String/Path?(string/path=w302) -> (empty?=w301:bool)
            n186 = property on="Class Name" class="Str"("Val(Sgnl)"=w303) -> ()  [unwired: 2 in, 2 out]
            n187 = case shown="False" w301 {
              tunnel: w300 -> [w342 _]
              frame False {
                n188 = Strip Path(path=w342) -> (stripped path=w341:path)  [unwired: 1 out]
                n189 = local write "ClassPath"(w341) -> ()
              }
              frame True {
              }
            }
            n190 = property on="Class owner" class="Ring (strict)"("Visible"=w298) -> ()  [unwired: 2 in, 2 out]
          }
          event Panel Close {
            n191 = event-data() -> ()  [unwired: 2 out]
          }
          event "Class Name": Value Change {
            n192 = event-data() -> ("OldVal"=w389:string)  [unwired: 2 out]
            n193 = local read "Class owner"() -> (w378:u16)
            n194 = local read "ClassPath"() -> (w388:path)
            n195 = local read "Stereo Type"() -> (w383:T1)
            n196 = call <resource>:"CommonVIs SterotypeStringParser.vi"("SterotypeStringIn"=w389) -> ("Name"=w367:string)  [unwired: 18 out]
            n197 = call <resource>:"CommonVIs SterotypeStringParser.vi"("SterotypeStringIn"="Class Name") -> ("Name"=w377:string)  [unwired: 18 out]
            n198 = Not A Number/Path/Refnum?(number/path/refnum=w388) -> (NaN/Path/Refnum?=w386:bool)
            n199 = Empty String/Path?(string/path=w388) -> (empty?=w387:bool)
            n200 = Or(x=w387, y=w386) -> (x .or. y?=w385:bool)
            n201 = call <resource>:"CommonVIs ClassItemStringParser.vi"("ClassItemNameIn"=w377) -> ("Name"=w374:string)  [unwired: 18 out]
            n202 = call <resource>:"CommonVIs ClassItemStringParser.vi"("ClassItemNameIn"=w367) -> ("Name"=w366:string)  [unwired: 18 out]
            n203 = To Lower Case(string=w374) -> (all lower case string=w365:string)
            n204 = Empty String/Path?(string/path=w365) -> (empty?=w364:bool)
            n205 = Empty String/Path?(string/path=w366) -> (empty?=w363:bool)
            n206 = Equal?(x=w383, y=T6."TYPE") -> (x = y?=w380:bool)
            n207 = Equal?(x=w383, y=T6."ENUM") -> (x = y?=w381:bool)
            n208 = Greater Than 0?(x=w378) -> (x > 0?=w379:bool)
            n209 = Search 1D Array(1D array=w375, element=w365) -> (index of element=w371:i32)  [unwired: 1 out]
            n210 = And(x=w364, y=w363) -> (x .and. y?=w362:bool)
            n211 = Greater Or Equal To 0?(x=w371) -> (x >= 0?=w373:bool)
            n212 = Or(x=w380, y=w381) -> (x .or. y?=w376:bool)
            n213 = Compound Arithmetic op=AND(w376, invert w379) -> (w368:bool)
            n214 = Compound Arithmetic op=AND(w373, invert w376) -> (w372:bool)
            n215 = case shown="False" w362 {
              tunnel: w388 -> [w400 _]
              tunnel: w385 -> [w399 _]
              tunnel: w383 -> [w398 _]
              tunnel: w374 -> [w397 _]
              tunnel: w372 -> [w396 _]
              tunnel: w371 -> [w395 _]
              tunnel: w370 -> [w394 _]
              tunnel: w369 -> [w393 _]
              tunnel: w368 -> [w392 _]
              tunnel: w366 -> [w391 _]
              frame False {
                n216 = case shown="False" w396 {
                  tunnel: w391 -> [w407 _]
                  tunnel: w400 -> [w406 _]
                  tunnel: w399 -> [w405 _]
                  tunnel: w398 -> [w404 _]
                  tunnel: w397 -> [w403 _]
                  tunnel: w395 -> [_ w418]
                  tunnel: w394 -> [_ w417]
                  tunnel: w393 -> [w402 _]
                  tunnel: w392 -> [w401 _]
                  frame False {
                    n217 = case shown="True" w405 {
                      tunnel: w404 -> [w415 _]
                      tunnel: w406 -> [w414 _]
                      tunnel: w403 -> [w409 _]
                      tunnel: w407 -> [w412 _]
                      tunnel: w402 -> [w410 _]
                      tunnel: w401 -> [w408 _]
                      frame False {
                        n218 = call <resource>:"GuessPathFromName.vi"("Don'tAppendName"=w408, "FolderSuffix"=w410, "NewName"=w409, "OldName"=w412, "Stereo Type"=w415, "PathIn"=w414) -> ("File Path"=w411:path)  [unwired: 5 in]
                        n219 = local write "ClassPath"(w411) -> ()
                        n220 = call <resource>:"UMLEditor_RelativePath.vi"("Path In"=w411) -> ("ConvertedToARelativePath"=w413:bool)  [unwired: 1 in, 17 out]
                        n221 = property on="RelText" class="Str"("Visible"=w413) -> ()  [unwired: 2 in, 2 out]
                      }
                      frame True {
                      }
                    }
                  }
                  frame True {
                    n222 = Index Array(array=w417, index=w418) -> (element=w416:path)
                    n223 = local write "ClassPath"(w416) -> ()
                  }
                }
              }
              frame True {
              }
            }
          }
          event "ClassPath": Value Change {
            n224 = event-data() -> ()  [unwired: 2 out]
            n225 = call <vilib>:"Get File Extension.vi"("file"="ClassPath") -> ("filename without extension"=w419:string, "lowercase file extension"=w420:string)  [unwired: 1 in, 8 out]
            n226 = case shown="Default" w420 {
              tunnel: w419 -> [_ w426 w433]
              frame Default {
                n227 = local read "Class Name"() -> (w425:string)
                n228 = property on="Class Name" class="Str"("Val(Sgnl)"=w425) -> ()  [unwired: 2 in, 2 out]
              }
              frame "ctl" {
                n229 = local read "Stereo Type"() -> (w430:T1)
                n230 = case shown="Default" w430 {
                  selector: w430 -> [_ w432]
                  tunnel: [w431 w432] -> w428
                  frame Default {
                    w431 = CommonVIs_StereoType."TYPE" ("Stereo Type")
                    n231 = local write "Stereo Type"(w431) -> ()
                  }
                  frame "TYPE", "ENUM" {
                  }
                }
                n232 = Format Into String(format string="<<%s>>\n%s", w428, w426) -> (resulting string=w427:string)  [unwired: 2 in, 1 out]
                n233 = local write "Class Name"(w427) -> ()
              }
              frame "vi", "vit" {
                n234 = local read "Stereo Type"() -> (w437:T1)
                n235 = case shown="Default" w437 {
                  selector: w437 -> [_ w439]
                  tunnel: [w438 w439] -> w435
                  frame Default {
                    w438 = CommonVIs_StereoType."VI" ("Stereo Type")
                    n236 = local write "Stereo Type"(w438) -> ()
                  }
                  frame "APPLICATION", "VI" {
                  }
                }
                n237 = Format Into String(format string="<<%s>>\n%s", w435, w433) -> (resulting string=w434:string)  [unwired: 2 in, 1 out]
                n238 = local write "Class Name"(w434) -> ()
              }
            }
            n239 = Empty String/Path?(string/path="ClassPath") -> (empty?=w422:bool)
            n240 = call <resource>:"UMLEditor_RelativePath.vi"("Path In"="ClassPath") -> ("ConvertedToARelativePath"=w423:bool)  [unwired: 1 in, 17 out]
            n241 = Compound Arithmetic op=AND(invert w422, w423) -> (w424:bool)
            n242 = property on="RelText" class="Str"("Visible"=w424) -> ()  [unwired: 2 in, 2 out]
          }
          event "Class owner": Value Change {
            n243 = event-data() -> ()  [unwired: 2 out]
            n244 = property on="Class owner" class="Ring (strict)"() -> ("Visible"=w440:bool)  [unwired: 2 in, 2 out]
            n245 = case shown="True" w440 {
              tunnel: w442 -> [_ w448]
              tunnel: "Class owner" -> [_ w447]
              frame False {
              }
              frame True {
                n246 = local read "Class Name"() -> (w457:string)
                n247 = property on="Class owner" class="Ring (strict)"() -> ("Strings []"=w453:string[])  [unwired: 2 in, 2 out]
                n248 = Index Array(array=w448, index=w447) -> (element=w443:path)
                n249 = Empty String/Path?(string/path=w443) -> (empty?=w446:bool)
                n250 = Not A Number/Path/Refnum?(number/path/refnum=w443) -> (NaN/Path/Refnum?=w445:bool)
                n251 = call <resource>:"CommonVIs SterotypeStringParser.vi"("SterotypeStringIn"=w457) -> ("Name"=w456:string, "Sterotype"=w455:string)  [unwired: 17 out]
                n252 = Index Array(array=w453, index=w447) -> (element=w452:string)
                n253 = Or(x=w446, y=w445) -> (x .or. y?=w444:bool)
                n254 = call <resource>:"CommonVIs ClassItemStringParser.vi"("ClassItemNameIn"=w456) -> ("Name"=w451:string)  [unwired: 18 out]
                n255 = case shown="True" w444 {
                  tunnel: w443 -> [w458 _]
                  frame False {
                    n256 = local write "ClassPath"(w458) -> ()
                  }
                  frame True {
                    n257 = disable-structure shown="Disabled" {
                      frame Disabled {
                        n258 = local write "ClassPath"(path "" ("ClassPath")) -> ()
                      }
                      frame Enabled {
                      }
                    }
                  }
                }
                n259 = case shown="Default" w455 {
                  selector: w455 -> [w471 _]
                  tunnel: [w472 _] -> w454
                  frame Default {
                    n260 = Format Into String(format string="<<%s>>\n", w471) -> (resulting string=w472:string)  [unwired: 2 in, 1 out]
                  }
                  frame "" {
                  }
                }
                n261 = case shown="\"\"" w451 {
                  selector: w451 -> [w460 _]
                  tunnel: [w460 "NewType"] -> w450
                  frame Default {
                  }
                  frame "" {
                  }
                }
                n262 = case shown="0, Default" w447 {
                  tunnel: w450 -> [w463 w469]
                  tunnel: w454 -> [w465 w468]
                  tunnel: [w462 w467] -> w449
                  tunnel: w452 -> [_ w466]
                  frame 0, Default {
                    n263 = Format Into String(format string="%s", initial string=w465, w463) -> (resulting string=w462:string)  [unwired: 1 in, 1 out]
                  }
                  frame 1.. {
                    n264 = Format Into String(format string="%s : %s", initial string=w468, w466, w469) -> (resulting string=w467:string)  [unwired: 1 in, 1 out]
                  }
                }
                n265 = property on="Class Name" class="Str"("Val(Sgnl)"=w449) -> ()  [unwired: 2 in, 2 out]
              }
            }
          }
          event "AddAttribute": Value Change {
            n266 = event-data() -> ()  [unwired: 4 out]
            n267 = local read "Attribute"() -> (w475:string)
            n268 = call <resource>:"AttributeGuide.vi"() -> ("Preview"=w474:string, "Canceled"=w476:bool)  [unwired: 18 out]
            n269 = case shown="False" w476 {
              tunnel: w475 -> [w482 _]
              tunnel: w474 -> [w479 _]
              frame False {
                n270 = call <vilib>:"Trim Whitespace.vi"("string"=w482) -> ("trimmed string"=w480:string)  [unwired: 1 in]
                n271 = Format Into String(format string="%s\n%s", w480, w479) -> (resulting string=w478:string)  [unwired: 2 in, 1 out]
                n272 = call <vilib>:"Trim Whitespace.vi"("string"=w478) -> ("trimmed string"=w477:string)  [unwired: 1 in]
                n273 = local write "Attribute"(w477) -> ()
              }
              frame True {
              }
            }
          }
          event "AddMethod": Value Change {
            n274 = event-data() -> ()  [unwired: 4 out]
            n275 = local read "Attribute"() -> (w489:string)
            n276 = local read "Methods"() -> (w492:string)
            n277 = call <vilib>:"Trim Whitespace.vi"("string"=w489) -> ("trimmed string"=w488:string)  [unwired: 1 in]
            n278 = Spreadsheet String To Array(delimiter (Tab)="\n", format string="%s", spreadsheet string=w488, array type (2D Dbl)=string[] [] ("Attributes")) -> (array=w484:string[])
            n279 = for {
              tunnel: w484 -> [w500] mode=indexing
              tunnel: [w496] -> w483 mode=indexing
              n280 = Match Pattern(string=w500, regular expression="^[\\s+#-]+") -> (before substring=w498:string, after substring=w497:string)  [unwired: 1 in, 2 out]
              n281 = Concatenate Strings(w498, w497) -> (w494:string)
              n282 = Match Pattern(string=w494, regular expression=":") -> (before substring=w493:string)  [unwired: 1 in, 3 out]
              n283 = call <vilib>:"Trim Whitespace.vi"("string"=w493) -> ("trimmed string"=w496:string)  [unwired: 1 in]
            }
            n284 = call <resource>:"MethodGuide.vi"("Attributes"=w483) -> ("Preview"=w491:string, "Canceled"=w490:bool)  [unwired: 17 out]
            n285 = case shown="False" w490 {
              tunnel: w492 -> [w506 _]
              tunnel: w491 -> [w503 _]
              frame False {
                n286 = call <vilib>:"Trim Whitespace.vi"("string"=w506) -> ("trimmed string"=w504:string)  [unwired: 1 in]
                n287 = Format Into String(format string="%s\n%s", w504, w503) -> (resulting string=w502:string)  [unwired: 2 in, 1 out]
                n288 = call <vilib>:"Trim Whitespace.vi"("string"=w502) -> ("trimmed string"=w501:string)  [unwired: 1 in]
                n289 = local write "Methods"(w501) -> ()
              }
              frame True {
              }
            }
          }
          event "Help": Value Change {
            n290 = event-data() -> ()  [unwired: 2 out]
            n291 = case shown="True" "Help" {
              tunnel: [ContextHelp_HelpTexts."None(Hide)" ("HelpText") ContextHelp_HelpTexts."Default" ("HelpText")] -> w508
              frame False {
              }
              frame True {
              }
            }
            n292 = call <resource>:"ContextHelp_HelpTexts.vi"("HelpText (enum or string)"=w508) -> ("HelpOut"=w509:T11)  [unwired: 18 out]
            n293 = call <resource>:"ContextHelp_SendMessageToPopUp.vi"("PopUpMessage"=w509) -> ()  [unwired: 2 in, 17 out]
          }
          event Mouse Enter {
            n294 = event-data() -> ("CtlRef"=w513:refnum<vi>)  [unwired: 1 out]
            n295 = local read "Help"() -> (w512:bool)
            n296 = call <resource>:"ContextHelp_CheckHelpForControl.vi"("Ctl Refnum"=w513, "Help"=w512) -> ()  [unwired: 1 in, 17 out]
          }
        }
      }
      n297 = call <resource>:"CommonVIs_CloseControlRefs.vi"("Event Registration Refnum"=w99, "ControlRefs"=w103) -> ("error out"=w102:errorcluster)  [unwired: 1 in, 16 out]
      n298 = case shown="True" w129 {
        tunnel: [w516 w555] -> w134
        tunnel: [w517 w554] -> w133
        tunnel: w15 -> [w517 w553]
        tunnel: w130 -> [_ w552]
        tunnel: w121 -> [_ w547]
        tunnel: w120 -> [_ w546]
        tunnel: w119 -> [w516 w545]
        tunnel: w37 -> [_ w541]
        tunnel: [enum16{"NA", "Connect", "DisConnect"}."NA" ("changeConnection") w542] -> w114
        tunnel: [TRUE ("Key Focus") FALSE ("Key Focus")] -> w113
        frame False {
        }
        frame True {
          w536 = u16 1 items=["None", "TYPE", "GUI", "SINGLETON", "SIGNAL", "BOUNDARY", "ENTITY", "CONTROL", "LEGACY"] ("StereoType")
          n299 = local read "Stereo Type"() -> (w537:T1)
          n300 = local read "Class Name"() -> (w525:string)
          n301 = local read "ClassPath"() -> (w524:path)
          n302 = call <vilib>:"Trim Whitespace.vi"("string"="Methods") -> ("trimmed string"=w538:string)  [unwired: 1 in]
          n303 = call <vilib>:"Trim Whitespace.vi"("string"="Attribute") -> ("trimmed string"=w539:string)  [unwired: 1 in]
          n304 = call-dynamic "setText.vi"("reference"=w546, "text"=w538, "error in (no error)"=w545) -> ("error out"=w548:errorcluster)  [unwired: 15 in, 1 out]
          n305 = call <vilib>:"Trim Whitespace.vi"("string"=w525) -> ("trimmed string"=w527:string)  [unwired: 1 in]
          n306 = Equal?(x=w537, y=w536) -> (x = y?=w534:bool)
          n307 = call-dynamic "setText.vi"("reference"=w547, "text"=w539, "error in (no error)"=w548) -> ("error out"=w550:errorcluster)  [unwired: 15 in, 1 out]
          n308 = Path To String(path=w524) -> (string=w530:string)
          n309 = File/Directory Info(path=w524) -> (directory=w529:bool)  [unwired: 1 in, 6 out]
          n310 = Empty String/Path?(string/path=w524) -> (empty?=w535:bool)
          n311 = call-dynamic "setText.vi"("reference"=w552, "text"=w527, "error in (no error)"=w550) -> ("error out"=w551:errorcluster)  [unwired: 15 in, 1 out]
          n312 = case shown="True" "connection" {
            tunnel: [enum16{"NA", "Connect", "DisConnect"}."NA" ("changeConnection") w576] -> w542
            tunnel: w541 -> [_ w577]
            frame False {
            }
            frame True {
              n313 = Select(t=enum16{"NA", "Connect", "DisConnect"}."DisConnect" ("changeConnection"), s=w577, f=enum16{"NA", "Connect", "DisConnect"}."Connect" ("changeConnection")) -> (s? t:f=w576:enum16{"NA", "Connect", "DisConnect"})
            }
          }
          n314 = case shown="True" w529 {
            tunnel: w524 -> [w566 w571]
            tunnel: [w561 w572] -> w528
            tunnel: w527 -> [_ w570]
            frame False {
              n315 = Strip Path(path=w566) -> (stripped path=w563:path, name=w565:string)
              n316 = Concatenate Strings(w565, ".ctl" ("string")) -> (w562:string)
              n317 = Build Path(base path=w563, name or relative path=w562) -> (appended path=w561:path)
            }
            frame True {
              n318 = call <resource>:"CommonVIs SterotypeStringParser.vi"("SterotypeStringIn"=w570) -> ("Name"=w568:string)  [unwired: 18 out]
              n319 = Concatenate Strings(w568, ".ctl" ("string")) -> (w567:string)
              n320 = Build Path(base path=w571, name or relative path=w567) -> (appended path=w572:path)
            }
          }
          n321 = Match Pattern(string=w530, regular expression="\\2E[Cc][Tt][Ll]$") -> (offset past match=w532:i32)  [unwired: 4 out]
          n322 = call <resource>:"ClassNode_GetAttributes.vi"("reference in"=w553, "OnlyGetDvrReference(False)"=TRUE, "error in (no error)"=w551) -> ("reference out"=w554:refnum<class "ClassNode.lvclass">, "DataRef"=w521:refnum<data-value>, "error out"=w555:errorcluster)  [unwired: 13 in, 1 out]
          n323 = Less Than 0?(x=w532) -> (x < 0?=w531:bool)
          n324 = Compound Arithmetic op=AND(w531, w534, invert w535) -> ()  [unwired: 1 out]
          n325 = Select(t=w528, s=FALSE, f=w524) -> (s? t:f=w526:path)
          n326 = call <resource>:"UMLEditor_RelativePath.vi"("Path In"=w526) -> ("ConvertToRelativePath(If possible)"=w520:path)  [unwired: 1 in, 17 out]
          n327 = in-place {
            in-place-border: w520 -> [w559]
            in-place-border: "ShowMethods" -> [w558]
            in-place-border: "ShowAttrib" -> [w557]
            n328 = in-place-dvr #1(w521) -> (w560:T9)  [unwired: 1 out]
            n329 = Bundle By Name(cluster=w560, "ClassPath"=w559, "showMethods"=w558, "showAttributes"=w557) -> (w556:T9)
            n330 = in-place-dvr #1(w556) -> ()  [unwired: 2 out]
          }
        }
      }
      n331 = property on="AddAttribute" class="Bool"("Visible"=w27) -> ()  [unwired: 2 in, 2 out]
      n332 = property on="UserText" class="Str"("Visible"=w25, "Value"=w26) -> ()  [unwired: 2 in, 2 out]
      n333 = call <resource>:"ContextHelp_LeavingDialog.vi"("error in (no error)"=w102) -> ()  [unwired: 2 in, 17 out]
      n334 = property on="Attribute" class="Str"("Caption.Text"=w24) -> ()  [unwired: 2 in, 2 out]
      n335 = Search 1D Array(1D array=w57, element=w20) -> (index of element=w60:i32)  [unwired: 1 out]
      n336 = Max & Min(x=w60, y=0) -> (max(x,y)=w58:i32)  [unwired: 1 out]
      n337 = property on="Class owner" class="Ring (strict)"("Strings []"=w57, "Val(Sgnl)"=w58) -> ()  [unwired: 2 in, 2 out]
    }
    frame Error {
    }
  }
  "reference out" <- w6
  "error out" <- w7
  "changeConnection" <- w4
  "cancel" <- w3
  "UserText" <- w2
